vi "Copy .LLB to NI VeriStand dir.vi"(5 "Files Generated by Build":path[](array[path]), 6 "Top Level/Always Included VIs":path[](array[path]), 7 "Destination Path":path, 8 "error in (no error)":errorcluster, 9 "Target Name":string, 10 "Build Specification Name":string, 11 "Project Path":path) -> (0 "error out":errorcluster)   [LabVIEW 2024]
doc: "This VI is called after each run of a build specification. The VI will copy the generated LLB (Engine or System Explorer) into the VeriStand Custom Device folder (...\\Documents\\National Instruments\\NI VeriStand 2013...)."
uses:
  <vilib>/Utility/sysdir.llb/System Directory Type.ctl
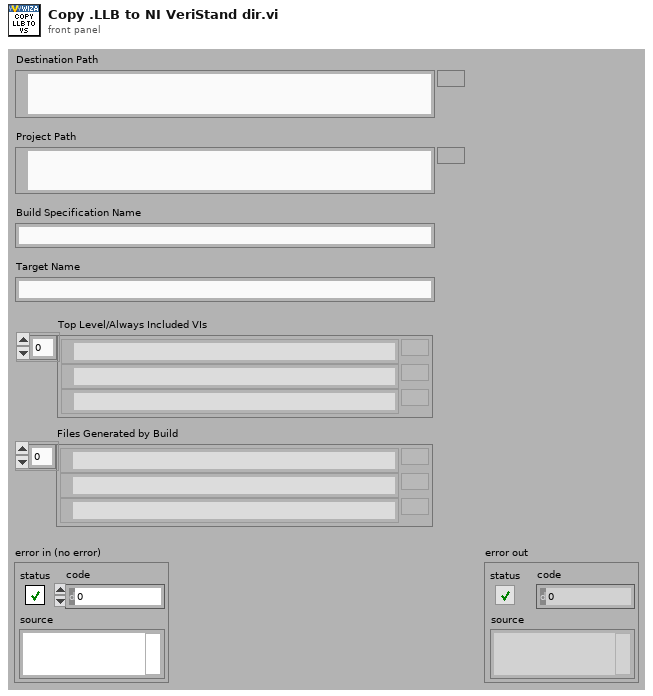
[diagram p1: front panel]
types:
  T1 = typedef "System Directory Type.ctl" = i32
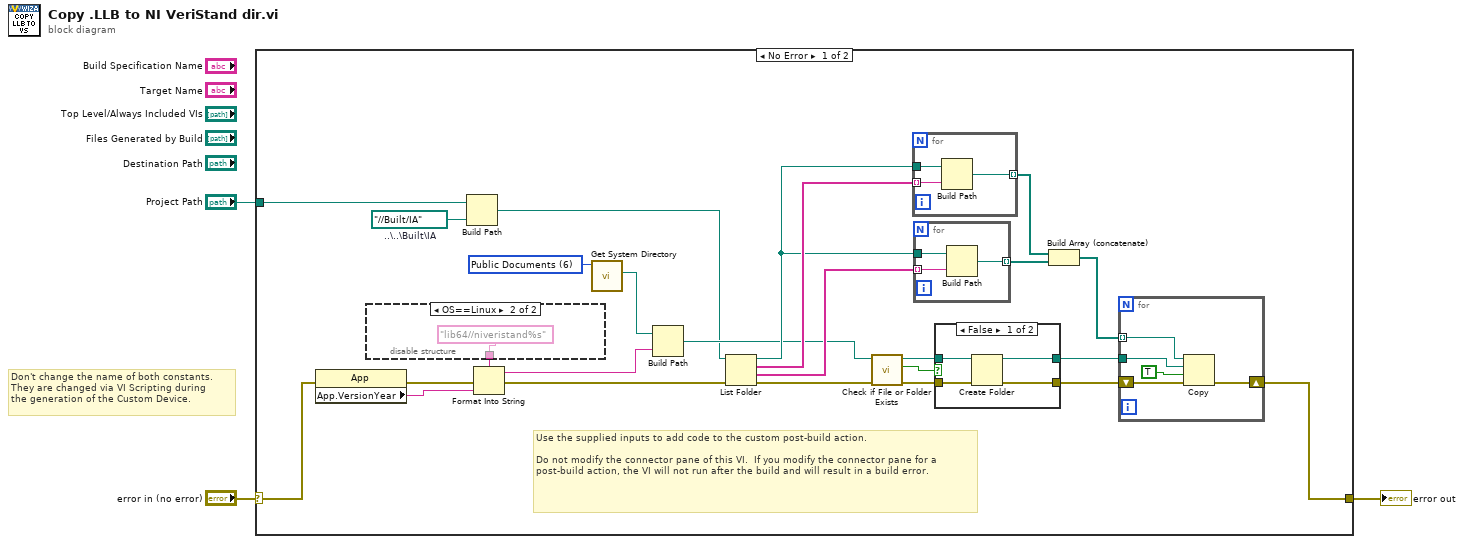
[diagram p0: block diagram]
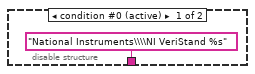
[diagram p2: hidden frame]
diagram:
  # "Don't change the name of both constants.\nThey are changed via VI Scripting during\nthe generation of the Custom Device."
  n1 = case shown="No Error" "error in (no error)" {
    selector: "error in (no error)" -> [w10 w48]
    tunnel: [w12 w48] -> w1
    tunnel: "Project Path" -> [w8 _]
    frame No Error {
      w4 = path "../../Built/IA"  # ..\..\Built\IA
      w16 = T1 6 items=["User Home"=0, "User Desktop"=1, "User Documents"=2, "User Application Data"=3, "User Preferences"=4, "User Temporary"=5, "Public Documents"=6, "Public Application Data"=7, "Public Preferences"=8, "Public Cache"=13, "System Core Libraries"=9, "System Installed Libraries"=10, "Application Files"=11, "Boot Volume Root"=12] ("system directory type")
      # "Use the supplied inputs to add code to the custom post-build action.\n\nDo not modify the connector pane of this VI.  If you modify the connector pane for a post-build action, the VI will not run after the build and will result in a build error."
      n2 = property class="App"(error in=w10) -> (error out=w15:errorcluster, "App.VersionYear"=w14:string)  [unwired: 1 in, 1 out]
      n3 = disable-structure shown="OS==Linux" {
        disable-tunnel: ["National Instruments\\\\NI VeriStand %s" ("name or relative path") "lib64//niveristand%s" ("name or relative path")] -> w13
        frame condition #0 (active) {
        }
        frame condition #1 {
        }
      }
      n4 = Build Path(base path=w8, name or relative path=w4) -> (appended path=w5:path)
      n5 = Format Into String(format string=w13, error in=w15, w14) -> (resulting string=w18:string, error out=w9:errorcluster)  [unwired: 1 in]
      n6 = call <vilib>:"Get System Directory.vi"("system directory type"=w16) -> ("system directory"=w17:path)  [unwired: 10 in]
      n7 = Build Path(base path=w17, name or relative path=w18) -> (appended path=w11:path)
      n8 = List Folder(path=w5, error in=w9) -> (path out=w21:path, filenames=w28:string[], folder names=w22:string[], error out=w19:errorcluster)  [unwired: 2 in]
      n9 = call <vilib>:"Check if File or Folder Exists.vi"("error in (no error)"=w19, "path"=w11) -> ("error out"=w23:errorcluster, "file or folder exists?"=w25:bool, "dup path"=w24:path)  [unwired: 7 in]
      n10 = for {
        tunnel: w28 -> [w46] mode=indexing
        tunnel: w21 -> [w47]
        tunnel: [w45] -> w27 mode=indexing
        n11 = Build Path(base path=w47, name or relative path=w46) -> (appended path=w45:path)
      }
      n12 = for {
        tunnel: w22 -> [w43] mode=indexing
        tunnel: w21 -> [w44]
        tunnel: [w42] -> w20 mode=indexing
        n13 = Build Path(base path=w44, name or relative path=w43) -> (appended path=w42:path)
      }
      n14 = case shown="False" w25 {
        tunnel: w24 -> [w34 w36]
        tunnel: w23 -> [w33 w35]
        tunnel: [w32 w36] -> w7
        tunnel: [w31 w35] -> w6
        frame False {
          n15 = Create Folder(path (use dialog)=w34, error in=w33) -> (created path=w32:path, error out=w31:errorcluster)  [unwired: 1 in, 1 out]
        }
        frame True {
        }
      }
      n16 = Build Array (concatenate)(w27, w20) -> (w26:path[])
      n17 = for {
        tunnel: w26 -> [w38] mode=indexing
        shift-right: [w39] -> w12
        shift-left: w6 -> [w40]
        tunnel: w7 -> [w37]
        n18 = Copy(8:w40, 9:TRUE ("overwrite (F)"), 10:w37, 11:w38) -> (0:w39:errorcluster)  [unwired: 1 in, 2 out]
      }
    }
    frame Error {
    }
  }
  "error out" <- w1
